vi "getOutputDAQ.vi"(8 "error in (no error)":errorcluster, 11 "Instrument.Lockin in":refnum<class "Instrument.Lockin.lvclass">) -> (0 "error out":errorcluster, 2 "OutputDAQ":T1, 3 "Instrument.Lockin out":refnum<class "Instrument.Lockin.lvclass">)   [LabVIEW 2019, in "Instrument.Lockin.lvlib" / "Instrument.Lockin.lvclass"]
doc: "API to configure DAQ settings.\n\nIf address=\"\", this API reads from localhost\nIf address is remote lockin, you need to add this computer to allowed whitelist on the lockin computer you are trying to access."
uses:
  Instrument.Lockin.lvclass
  Lockin.Typedefs/DAQ/DAQ.Config.AO--Cluster--Array.ctl
  Lockin.Typedefs/DAQ/DAQ.Config.AO--Cluster.ctl
  Lockin.Typedefs/DAQ/DAQ.Config.AO.Range--enum.ctl
  Lockin.Typedefs/DAQ/DAQ.TerminalConfiguration--enum.ctl
  Lockin.Typedefs/API/Lockin.Commands--Enum.ctl
  0da4648c-bad1-415e-8ea2-da0aa7c6013a.vi
  <vilib>/PRIrvin/JSON-RPC/API/JSON to Variant.vi
  <vilib>/Utility/Data Type/Get Type Information.vi
  <vilib>/JDP Science/JSONtext/JSON type.vi
  <vilib>/JDP Science/JSONtext/Get Array Elements.vi
  <vilib>/JDP Science/JSONtext/JSON text to Variant.vi
  Lockin.Typedefs/Lockin.Typedefs.lvlib
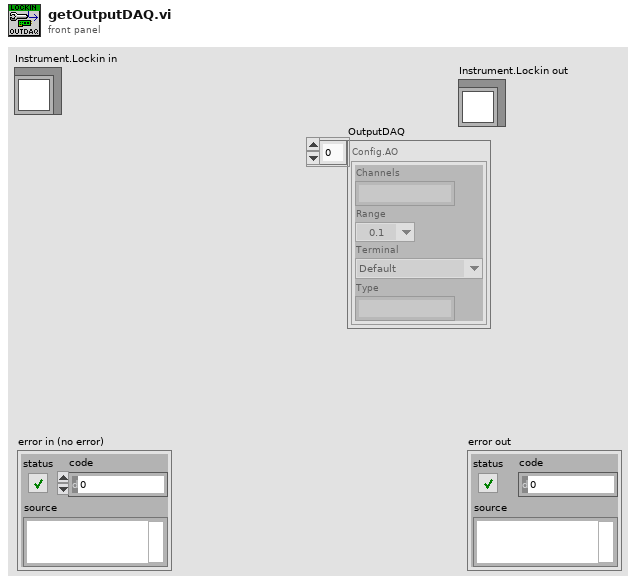
[diagram p1: front panel]
types:
  T1 = typedef "Lockin.Typedefs.lvlib/DAQ.Config.AO--Cluster--Array.ctl" = T2[]
  T2 = typedef "Lockin.Typedefs.lvlib/DAQ.Config.AO--Cluster.ctl" = cluster{"Channels":string, "Range":T3, "Terminal":T4, "Type":string}
  T3 = typedef "Lockin.Typedefs.lvlib/DAQ.Config.AO.Range--enum.ctl" = enum16{"0.1", "1.0", "3.5", "10.0", ""}
  T4 = typedef "Lockin.Typedefs.lvlib/DAQ.TerminalConfiguration--enum.ctl" = enum16{"Default", "Differential", "Pseudodifferential", ""}
  T5 = typedef "Lockin.Typedefs.lvlib/Lockin.Commands--Enum.ctl" = enum16{"setAO", "setAO_Amplitude", "setAO_DC", "setAO_Frequency", "setAO_Phase", "setAO_Function", "setREF", "setREF_Frequency", "setREF_Phase", "setREF_TC", "setREF_Roll-Off", "setDAQ", "setSampling", "setState", "getState", "getAO", "getAI", "getResults", "getSampling", "getAOconfig", "getREFconfig", "setInputGain", "setOutputGain", "getInputGain", "getOutputGain", "setSweep", "setSweepTime", "setSweepTable", "getStatus", "getSweepResults", "getSweepWaveforms", "logConfiguration", "startLogging", "stopLogging", "setInputOffset", "getInputOffset", "setOutputOffset", "getOutputOffset", "getInputDAQ", "getOutputDAQ", "getLinkFrequency", "setLinkFrequency", "measureInputOffset", "getDevices"}
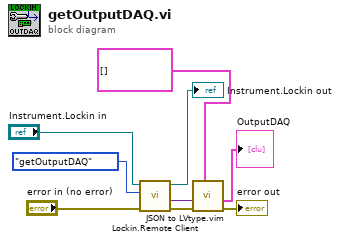
[diagram p0: block diagram]
diagram:
  n1 = call "Lockin.Remote Client.vi"("error in (no error)"="error in (no error)", "Command"=Lockin.Commands--Enum."getOutputDAQ" ("Enum"), "Instrument.Lockin in"="Instrument.Lockin in") -> ("error out"=w4:errorcluster, "Data out"=w5:variant, "Instrument.Lockin out"=→"Instrument.Lockin out":refnum<class "Instrument.Lockin.lvclass">)  [unwired: 6 in]
  n2 = call "JSON to LVtype.vim"("type"=T1 [] ("Config.AO []"), "error in (no error)"=w4, "JSON Data in"=w5) -> ("error out"=→"error out":errorcluster, "Data out"=→"OutputDAQ":T1)  [unwired: 7 in]
